vi "save Screenshot File.vi"(8 "error in (no error)":errorcluster, 10 "File Path":path, 11 "FSV-40N in":refnum<class "FSV-40N.lvclass">) -> (0 "error out":errorcluster, 3 "FSV-40N out":refnum<class "FSV-40N.lvclass">)   [LabVIEW 2023, in "Spectrum Analyzer.lvlib" / "FSV-40N.lvclass"]
uses:
  FSV-40N.lvclass
  FSV-40N.lvclass/FSV-40N.ctl
  Spectrum Analyzer.lvlib
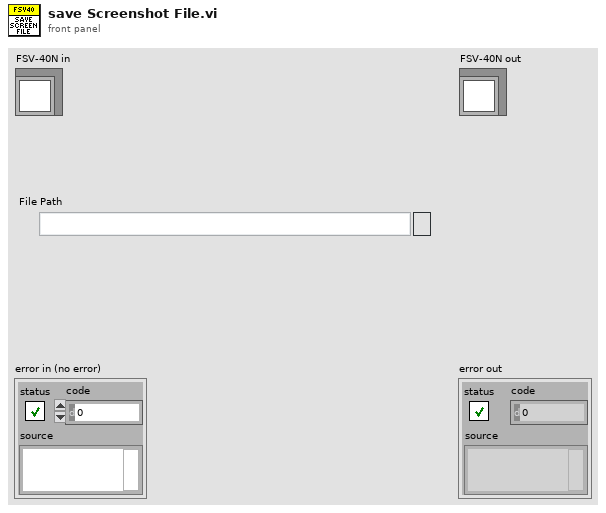
[diagram p1: front panel]
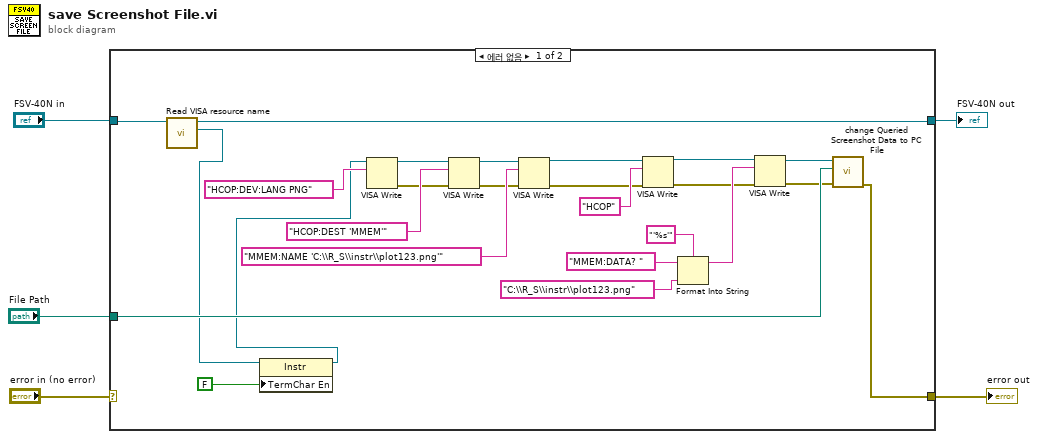
[diagram p0: block diagram]
diagram:
  n1 = case shown="에러 없음" "error in (no error)" {
    selector: "error in (no error)" -> [_ w31]
    tunnel: "FSV-40N in" -> [w30 w32]
    tunnel: [w21 w32] -> w3
    tunnel: [w12 w31] -> w2
    tunnel: "File Path" -> [w15 _]
    frame No Error {
      n2 = call "Read VISA resource name.vi"("FSV-40N in"=w30) -> ("VISA resource name"=w8:refnum<visa-resource-name>, "FSV-40N out"=w21:refnum<class "FSV-40N.lvclass">)  [unwired: 8 in, 1 out]
      n3 = property class="Instr"(reference=w8, "TermChar En"=FALSE ("Message Based Settings:Termination Character Enable")) -> (reference out=w6:refnum<visa-resource-name>)  [unwired: 1 in, 1 out]
      n4 = VISA Write(VISA resource name=w6, write buffer="HCOP:DEV:LANG PNG") -> (VISA resource name out=w22:refnum<visa-resource-name>, error out=w10:errorcluster)  [unwired: 1 in, 1 out]
      n5 = VISA Write(VISA resource name=w22, write buffer="HCOP:DEST 'MMEM'", error in (no error)=w10) -> (VISA resource name out=w25:refnum<visa-resource-name>, error out=w9:errorcluster)  [unwired: 1 out]
      n6 = VISA Write(VISA resource name=w25, write buffer="MMEM:NAME 'C:\\R_S\\instr\\plot123.png'" ("Name (\"D:\\output\")"), error in (no error)=w9) -> (VISA resource name out=w27:refnum<visa-resource-name>, error out=w26:errorcluster)  [unwired: 1 out]
      n7 = VISA Write(VISA resource name=w27, write buffer="HCOP", error in (no error)=w26) -> (VISA resource name out=w20:refnum<visa-resource-name>, error out=w14:errorcluster)  [unwired: 1 out]
      n8 = Format Into String(format string="'%s'", initial string="MMEM:DATA? ", "C:\\R_S\\instr\\plot123.png" ("Name (\"D:\\output\")")) -> (resulting string=w17:string)  [unwired: 1 in, 1 out]
      n9 = VISA Write(VISA resource name=w20, write buffer=w17, error in (no error)=w14) -> (VISA resource name out=w16:refnum<visa-resource-name>, error out=w13:errorcluster)  [unwired: 1 out]
      n10 = call "change Queried Screenshot Data to PC File.vi"("error in"=w13, "File Path"=w15, "VISA resource name In"=w16) -> ("error out"=w12:errorcluster)  [unwired: 7 in, 1 out]
    }
    frame Error {
    }
  }
  "error out" <- w2
  "FSV-40N out" <- w3
